vi "EPC300X Read From Register - Floating Point.vi"(7 "Unit Address (1)":u8=1, 8 "error in (no error)":errorcluster, 9 "Num Of Reg (1)":u16=1 min=1 step=1, 10 "Register Address (0)":u16, 11 "VISA session":refnum<visa-resource-name>) -> (0 "error out":errorcluster, 1 "Data (ms)":u32[](array[numeric]), 2 "Data (SGL)":sgl[](array[numeric]) format="%.3f", 3 "dup VISA session":refnum<visa-resource-name>, 4 "Read Buffer":u8[][](array[numeric]), 5 "Data 2 (U16)":u16[][](array[numeric]))   [LabVIEW 2022 SP3]
doc: "This VI reads value from specified registers of specified unit."
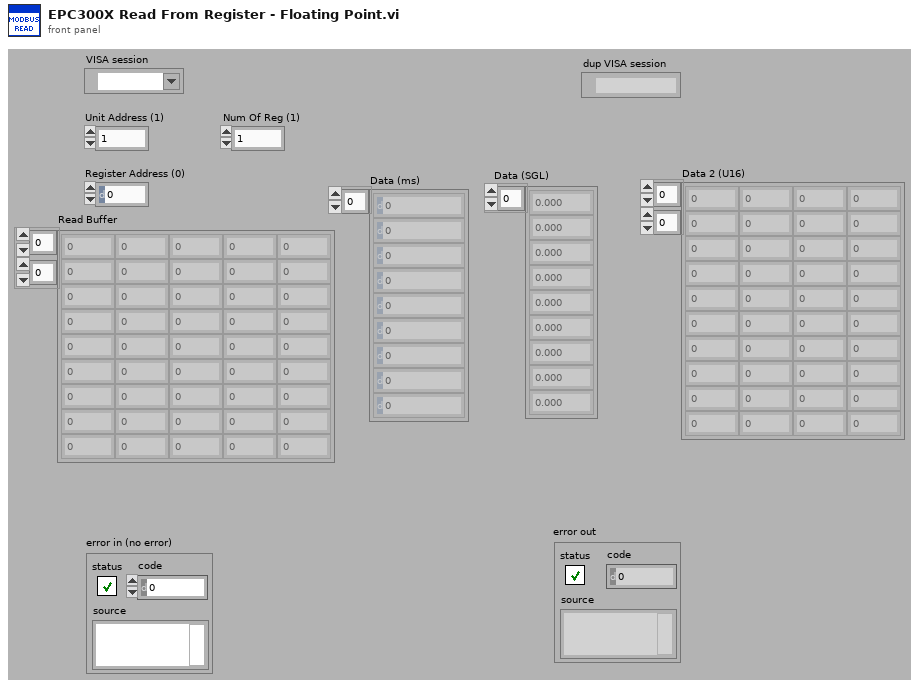
[diagram p1: front panel]
types:
  T1 = enum16{"By The Number of Bytes", "Copy Of the Sent Message"}
  T2 = cluster{"Read Buffer[0]":u8, "Read Buffer[1]":u8}
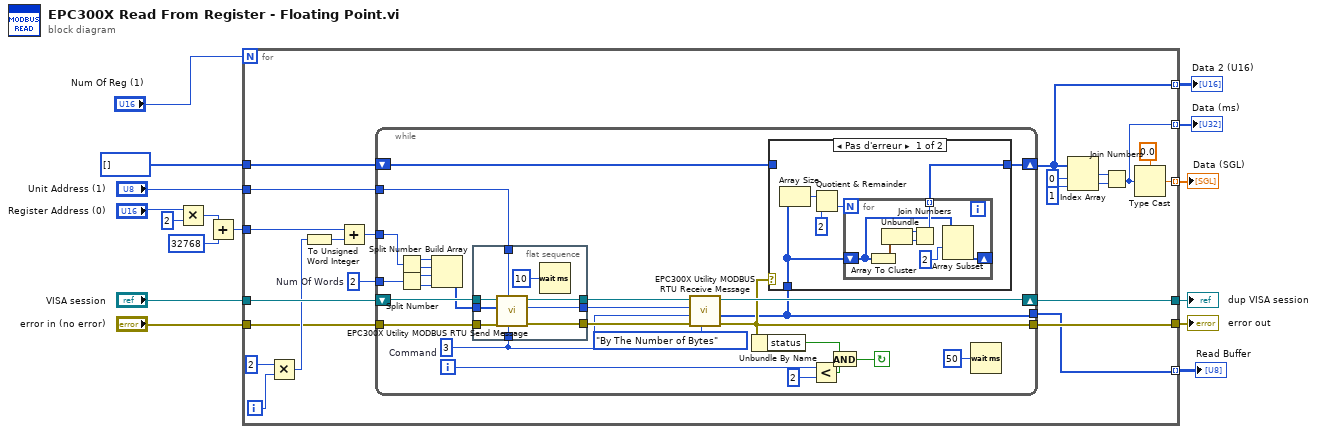
[diagram p0: block diagram]
diagram:
  n1 = Multiply(x="Register Address (0)", y=u16 2) -> (x*y=w9:u16)
  n2 = Add(x=w9, y=u16 32768) -> (x+y=w4:u16)
  n3 = for {
    N: "Num Of Reg (1)" -> [_]
    tunnel: "VISA session" -> [w38]
    tunnel: [w37] -> w15
    tunnel: u16[] [] -> [w36]
    tunnel: "error in (no error)" -> [w21]
    tunnel: [w20] -> w12
    tunnel: "Unit Address (1)" -> [w35]
    tunnel: w4 -> [w26]
    tunnel: [w28] -> w5 mode=indexing
    tunnel: [w19] -> w3 mode=indexing
    tunnel: [w18] -> w2 mode=indexing
    tunnel: [w17] -> w1 mode=indexing
    i -> [w25]
    w34 = u16 2  # Num Of Words
    n4 = Multiply(x=2, y=w25) -> (x*y=w23:i32)
    n5 = To Unsigned Word Integer(number=w23) -> (unsigned 16bit integer=w22:u16)
    n6 = Add(x=w26, y=w22) -> (x+y=w27:u16)
    n7 = while {
      tunnel: w35 -> [w46]
      shift-right: [w61] -> w37
      shift-left: w38 -> [w62]
      tunnel: w34 -> [w49]
      shift-right: [w51] -> w17
      shift-left: w36 -> [w50]
      tunnel: w27 -> [w42]
      tunnel: w21 -> [w41]
      tunnel: [w40] -> w20
      tunnel: [w39] -> w18
      i -> [w57]
      stop <- w59 continue-if-true
      w58 = u8 3  # Command
      n8 = Split Number(x=w42) -> (hi(x)=w53:u8, lo(x)=w52:u8)
      n9 = Split Number(x=w49) -> (hi(x)=w48:u8, lo(x)=w47:u8)
      n10 = Build Array(w53, w52, w48, w47) -> (w54:u8[])
      n11 = flat-sequence {
        tunnel: [w73] -> w64
        tunnel: [w72] -> w63
        tunnel: w62 -> [w71]
        tunnel: w58 -> [w70]
        tunnel: w54 -> [w69]
        tunnel: w46 -> [w68]
        tunnel: [w67] -> w44
        tunnel: w41 -> [w66]
        frame #0 {
          n12 = call "EPC300X Utility MODBUS RTU Send Message.vi"("Command (0)"=w70, "Unit Address (1)"=w68, "error in (no error)"=w66, "Message (empty array)"=w69, "VISA session"=w71) -> ("error out"=w73:errorcluster, "Length Of Sent MSG"=w67:u8, "dup VISA session"=w72:refnum<visa-resource-name>)  [unwired: 4 in]
          n13 = Wait (ms)(milliseconds to wait=u32 10) -> ()  [unwired: 1 out]
        }
      }
      n14 = call "EPC300X Utility MODBUS RTU Receive Message.vi"("Receive Message Type (0: By The Number Of Bytes)"=T1."By The Number of Bytes" ("Receive Message Type"), "error in (no error)"=w64, "Sent Command (0)"=w58, "Length Of Sent MSG (0)"=w44, "VISA session"=w63) -> ("error out"=w40:errorcluster, "Read Buffer"=w39:u8[], "dup VISA session"=w61:refnum<visa-resource-name>)  [unwired: 4 in]
      n15 = Unbundle By Name(w40) -> ("status"=w60:bool)
      n16 = case shown="Pas d'erreur" w40 {
        tunnel: w39 -> [w78 _]
        tunnel: [w77 w86] -> w51
        tunnel: w50 -> [_ w86]
        frame No Error {
          n17 = Array Size(array=w78) -> (size(s)=w76:i32)
          n18 = Quotient & Remainder(x=w76, y=2) -> (floor(x/y)=w74:i32)  [unwired: 1 out]
          n19 = for {
            N: w74 -> [_]
            shift-right: [w80] -> _
            shift-left: w78 -> [w81]
            tunnel: [w82] -> w77 mode=indexing
            n20 = Array To Cluster(array=w81) -> (cluster=w85:T2)
            n21 = Unbundle(w85) -> ("Read Buffer[0]"=w83:u8, "Read Buffer[1]"=w84:u8)
            n22 = Join Numbers(hi=w83, lo=w84) -> ((hi.lo)=w82:u16)
            n23 = Array Subset(array=w81, index=2) -> (w80:u8[])  [unwired: 1 in]
          }
        }
        frame Error {
        }
      }
      n24 = Less?(x=w57, y=2) -> (x < y?=w56:bool)
      n25 = And(x=w60, y=w56) -> (x .and. y?=w59:bool)
      n26 = Wait (ms)(milliseconds to wait=u32 50) -> ()  [unwired: 1 out]
    }
    n27 = Index Array(array=w17, index #1=0 ("index"), index #2=1 ("index")) -> (element #1=w32:u16, element #2=w33:u16)
    n28 = Join Numbers(hi=w32, lo=w33) -> ((hi.lo)=w19:u32)
    n29 = Type Cast(type=sgl 0.0, x=w19) -> (*(type *) &x=w28:sgl)
  }
  "error out" <- w12
  "dup VISA session" <- w15
  "Data (SGL)" <- w5
  "Data (ms)" <- w3
  "Read Buffer" <- w2
  "Data 2 (U16)" <- w1
